vi "Autonomous Independent.vi"() -> ()   [LabVIEW 2020]
doc: "This VI is called when autonomous begins, and will automatically be terminated when autonomous ends. You can carry out timed or sensor driven robot movement independently without needing to return to the caller."
uses:
  <vilib>/Rock Robotics/WPI/ThirdParty/REV Robotics/REVLib/Typedef/Spark MAX Sensor Type.ctl
  <vilib>/Rock Robotics/WPI/Solenoid/WPI_SolenoidValue.ctl
  <vilib>/Rock Robotics/WPI/Utilities/WPI_GetSetVariantRefNum.vi
  <vilib>/Rock Robotics/Network Tables/NT Read String.vi
  <vilib>/Rock Robotics/Network Tables/NT Write Numeric Array.vi
  <vilib>/Rock Robotics/Network Tables/NT Write Number.vi
  Robot Global Data.vi
  <vilib>/Rock Robotics/WPI/Solenoid/WPI_SolenoidSetEnum.vi
  <vilib>/Rock Robotics/WPI/RobotDrive/WPI_RobotDriveArcadeDrive_Standard(NoSaturation).vi
panel:
  out "Right Drive Encoder 2":dbl format="%#.3f"
  out "Sensor Position 2":dbl
  out "Timestamp 2":u32
  out "Sensor Position":dbl
  out "Timestamp":u32
  in  "error in 2":errorcluster
  out "Real Yaw":dbl
  out "Right Drive Encoder":dbl format="%#.3f"
  in  "error in":errorcluster
  # "Be sure to right-click and choose Data Operations>>Make Current Value default if you want to save the array values with the VI"
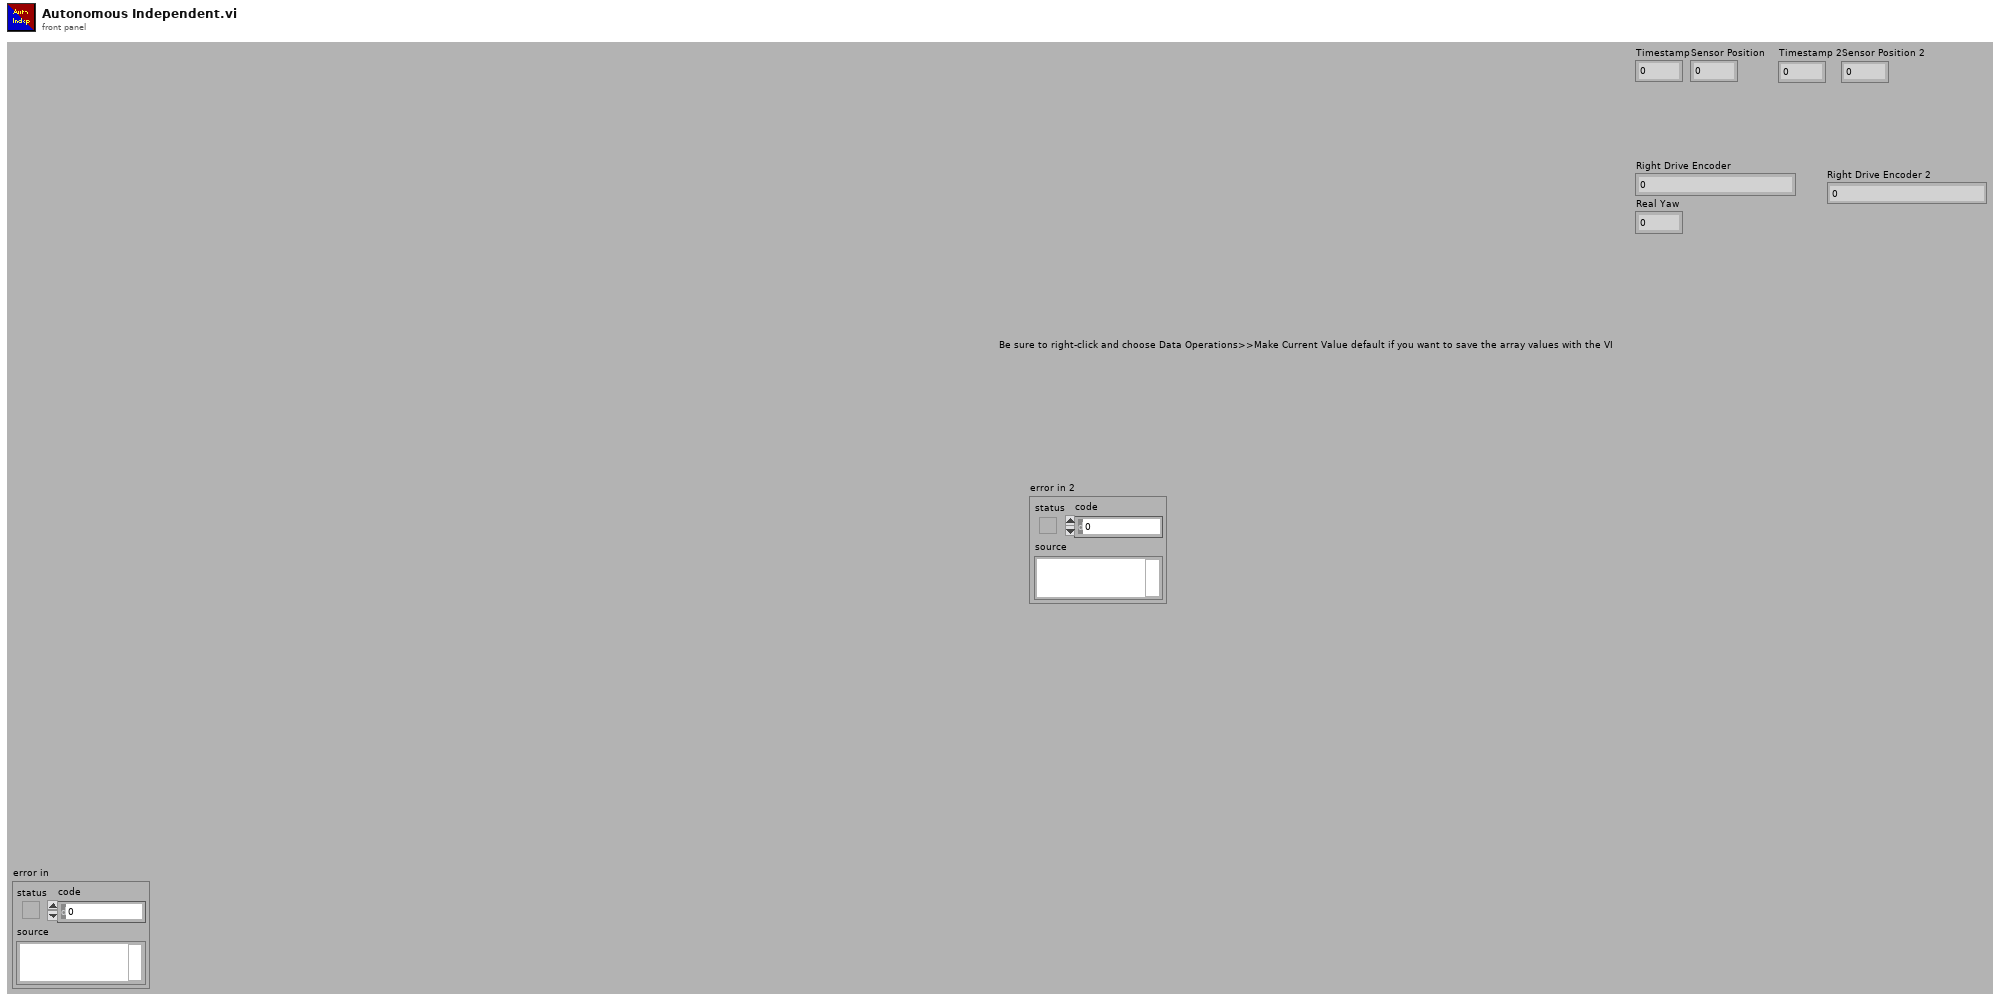
[diagram p1: front panel]
types:
  T1 = typedef "Spark MAX Sensor Type.ctl" = enum16{"No Sensor", "Hall Sensor", "Encoder", "-Not Available-", "Analog", "Alternate Encoder", "Duty Cycle"}
  T2 = typedef "WPI_JoystickDevRef.ctl" = cluster{"Device":T3}
  T3 = typedef "WPI_JoystickDeviceEnum.ctl" = enum16{"USB 0", "USB 1", "USB 2", "USB 3", "USB 4", "USB 5"}
  T4 = typedef "WPI_RobotDriveDevRef.ctl" = cluster{"DevStatus":errorcluster, "Motors[]":T5[], "Square Inputs":bool, "Max Output":dbl}
  T5 = typedef "WPI_MotorControlDeviceRef.ctl" = cluster{"DeviceStatus":errorcluster, "Type":T6, "PWM":cluster{"PWM Channel":T7, "DeadBand":T8}, "CAN":cluster{"Device Number":u8, "SetOutput VI Ref":variant, "GetOutput VI Ref":variant, "Enable VI Ref":variant, "Disable VI Ref":variant, "Data":variant}, "Invert":bool, "DIO PWM":cluster{"PWM \"Enable\" Channel":T7, "DIOChannel":T9, "PWM Rate":dbl}}
  T6 = typedef "WPI_MotorControlType.ctl" = enum16{"PWM", "CAN", "DIO PWM"}
  T7 = typedef "FPGA_DIOPWMChannel.ctl" = enum8{"PWM 0", "PWM 1", "PWM 2", "PWM 3", "PWM 4", "PWM 5", "PWM 6", "PWM 7", "PWM 8", "PWM 9", "PWM MXP 0", "PWM MXP 1", "PWM MXP 2", "PWM MXP 3", "PWM MXP 4", "PWM MXP 5", "PWM MXP 6", "PWM MXP 7", "PWM MXP 8", "PWM MXP 9", "Invalid"}
  T8 = typedef "WPI_PWMDeadband.ctl" = cluster{"Name":string, "maxPositivePwm":i32, "minPositivePwm":i32, "centerPwm":i32, "maxNegativePwm":i32, "minNegativePwm":i32, "angularRange":u16}
  T9 = typedef "FPGA_DIOChannel.ctl" = enum8{"DIO 0", "DIO 1", "DIO 2", "DIO 3", "DIO 4", "DIO 5", "DIO 6", "DIO 7", "DIO 8", "DIO 9", "DIO MXP 0", "DIO MXP 1", "DIO MXP 2", "DIO MXP 3", "DIO MXP 4", "DIO MXP 5", "DIO MXP 6", "DIO MXP 7", "DIO MXP 8", "DIO MXP 9", "DIO MXP 10", "DIO MXP 11", "DIO MXP 12", "DIO MXP 13", "DIO MXP 14", "DIO MXP 15", "SPI Port CS1", "SPI Port CS2", "SPI Port CS3", "SPI Port MISO", "SPI Port MOSI", "Invalid"}
  T10 = cluster{"Motors[][0]":T5, "Motors[][1]":T5, "Motors[][2]":T5, "Motors[][3]":T5, "Motors[][4]":T5, "Motors[][5]":T5, "Motors[][6]":T5, "Motors[][7]":T5, "Motors[][8]":T5}
  T11 = typedef "WPI_SolenoidValue.ctl" = enum16{"Off", "On", "Forward", "Reverse"}
  T12 = typedef "WPI_SolenoidDevRef.ctl" = cluster{"DevStatus":errorcluster, "Pneumatics Control Module":u8, "Forward Solenoid Channel":T13, "Reverse Solenoid Channel":T13}
  T13 = typedef "WPI_SolenoidChannel.ctl" = enum8{"Solenoid 0", "Solenoid 1", "Solenoid 2", "Solenoid 3", "Solenoid 4", "Solenoid 5", "Solenoid 6", "Solenoid 7", "Solenoid 8", "Solenoid 9", "Solenoid 10", "Solenoid 11", "Solenoid 12", "Solenoid 13", "Solenoid 14", "Solenoid 15", "Invalid"}
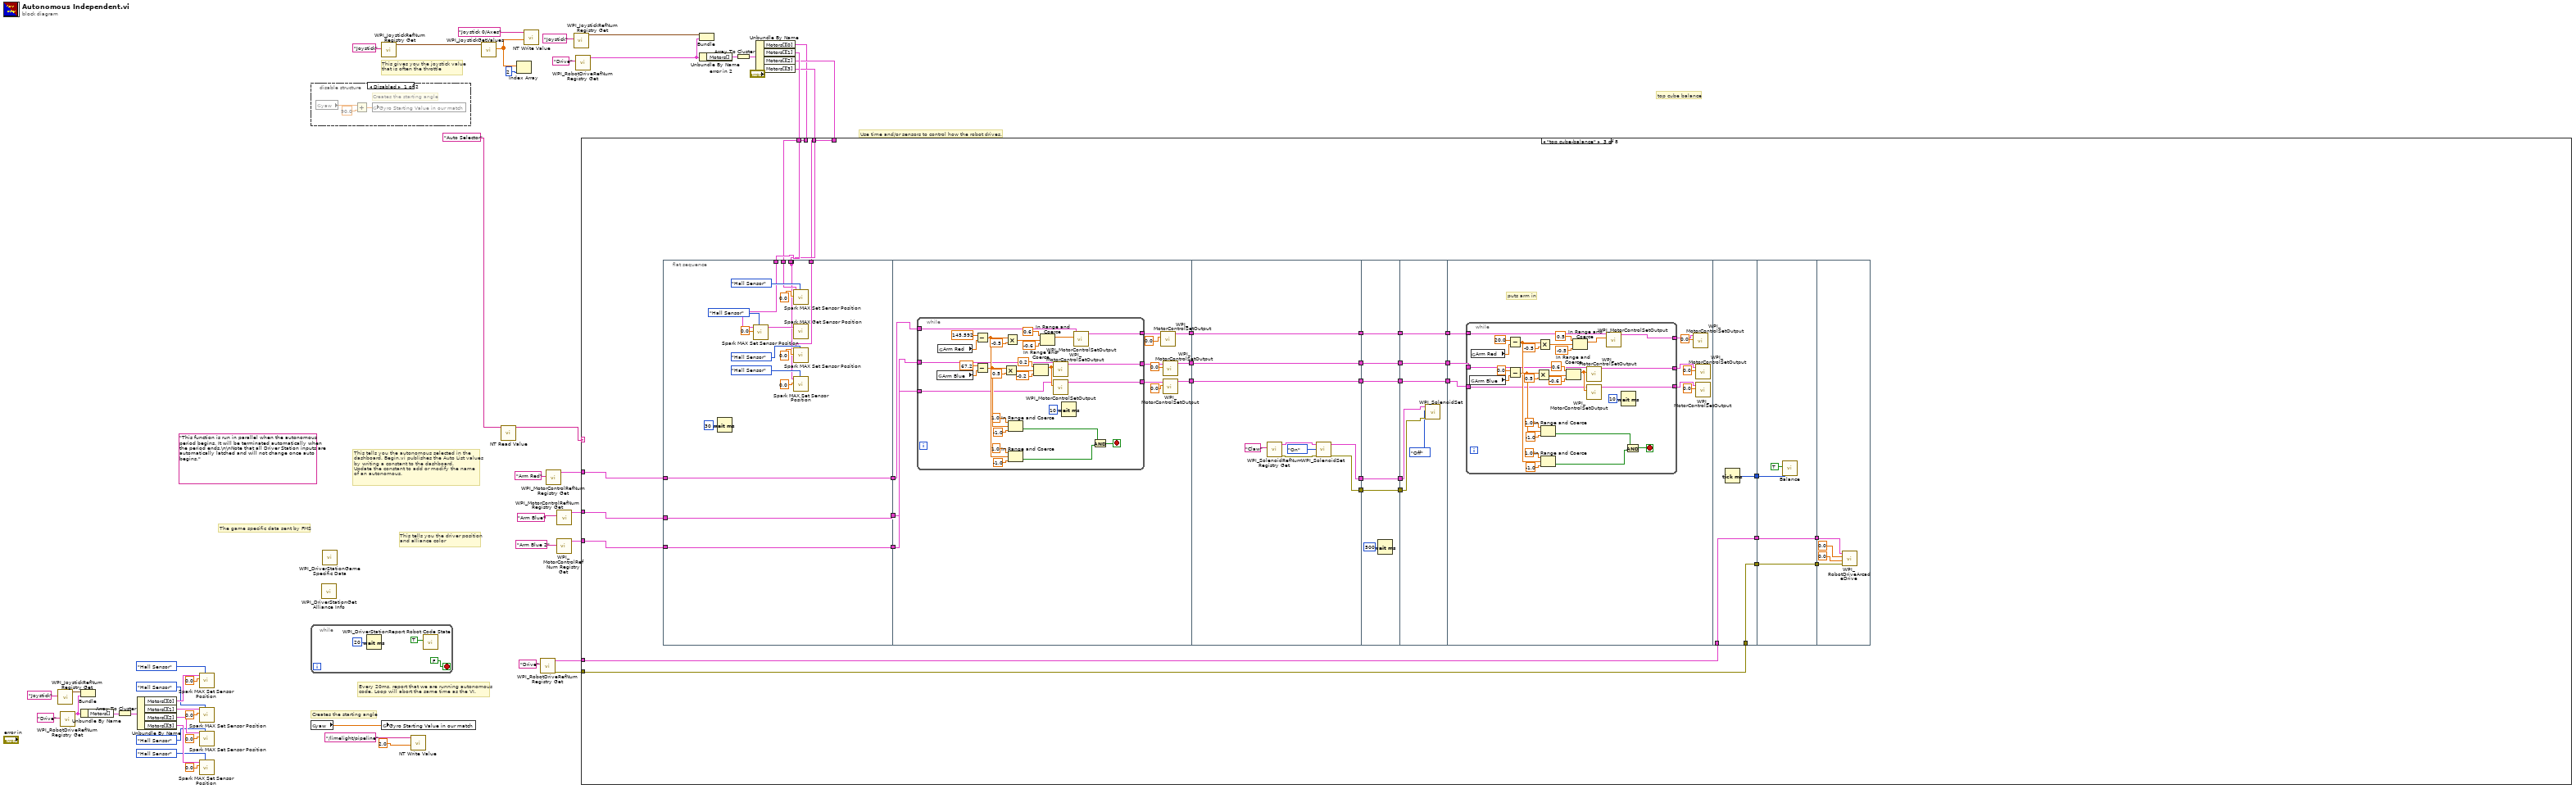
[diagram p0: block diagram]
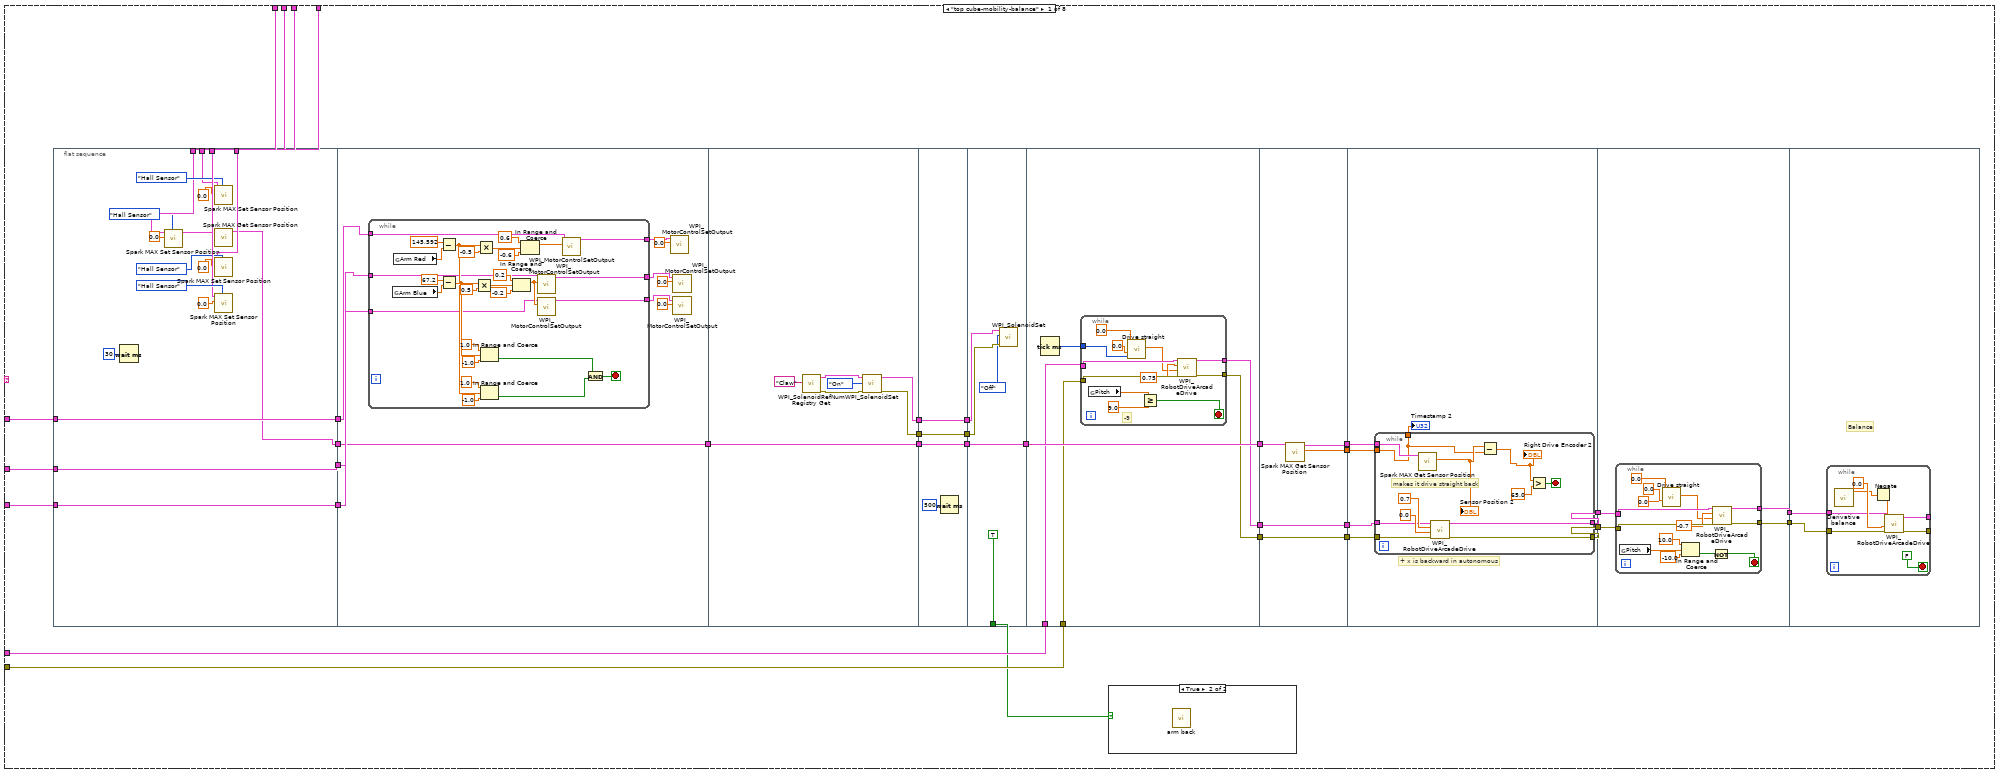
[diagram p3: hidden frame]
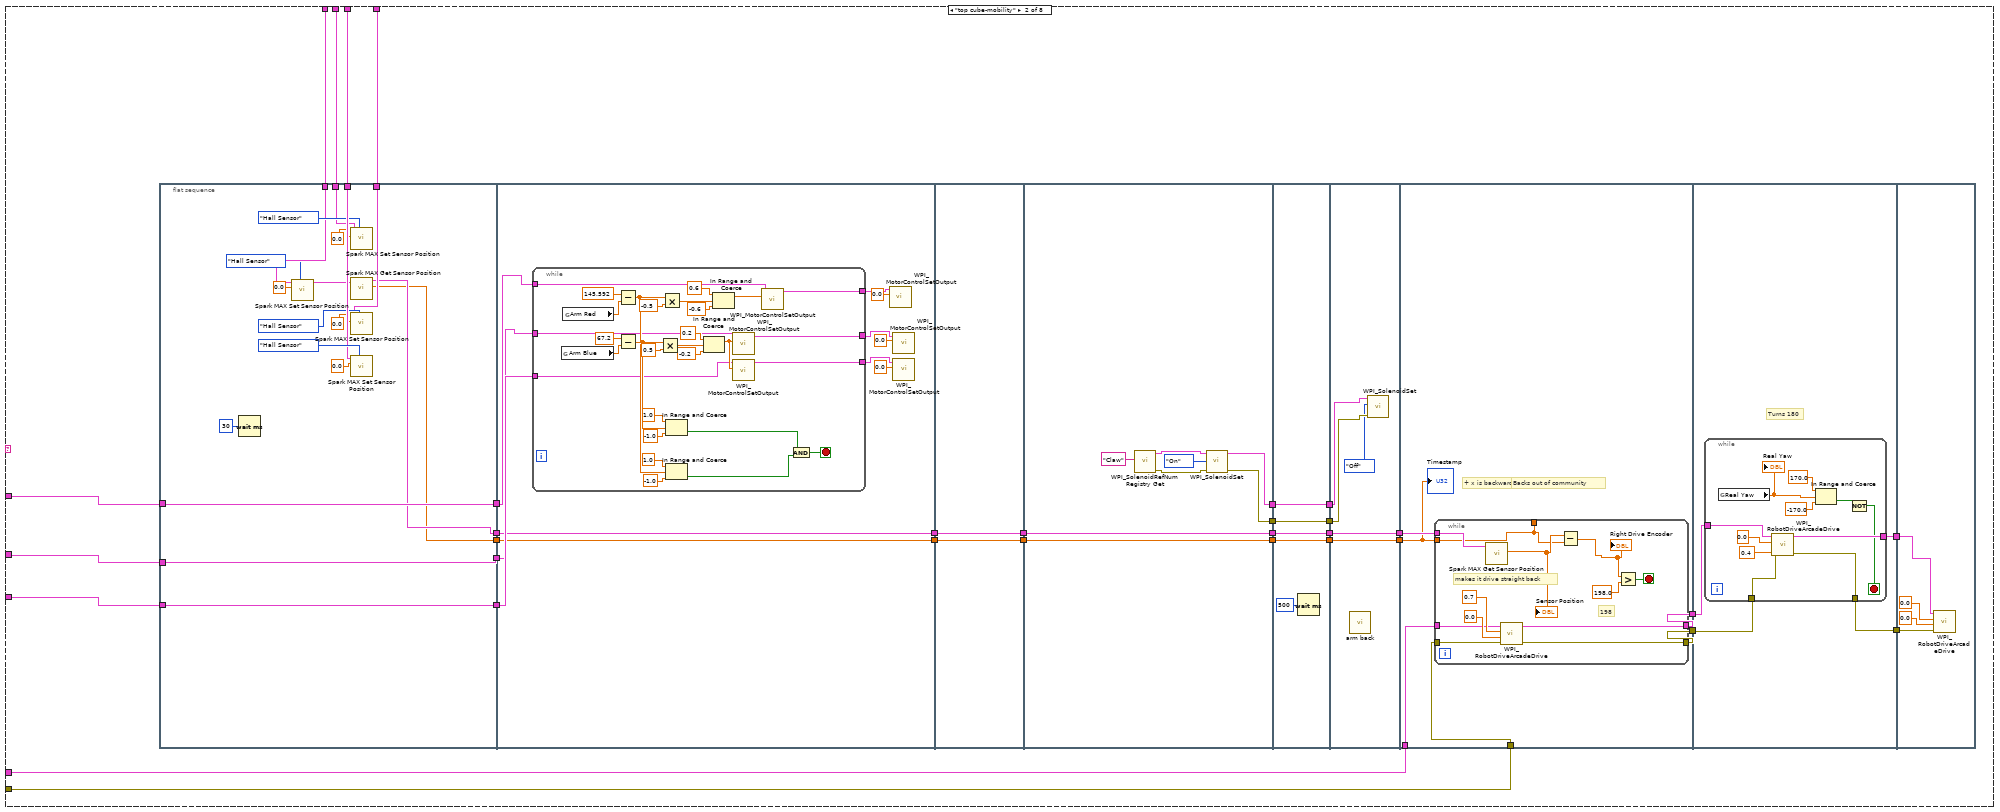
[diagram p5: hidden frame]
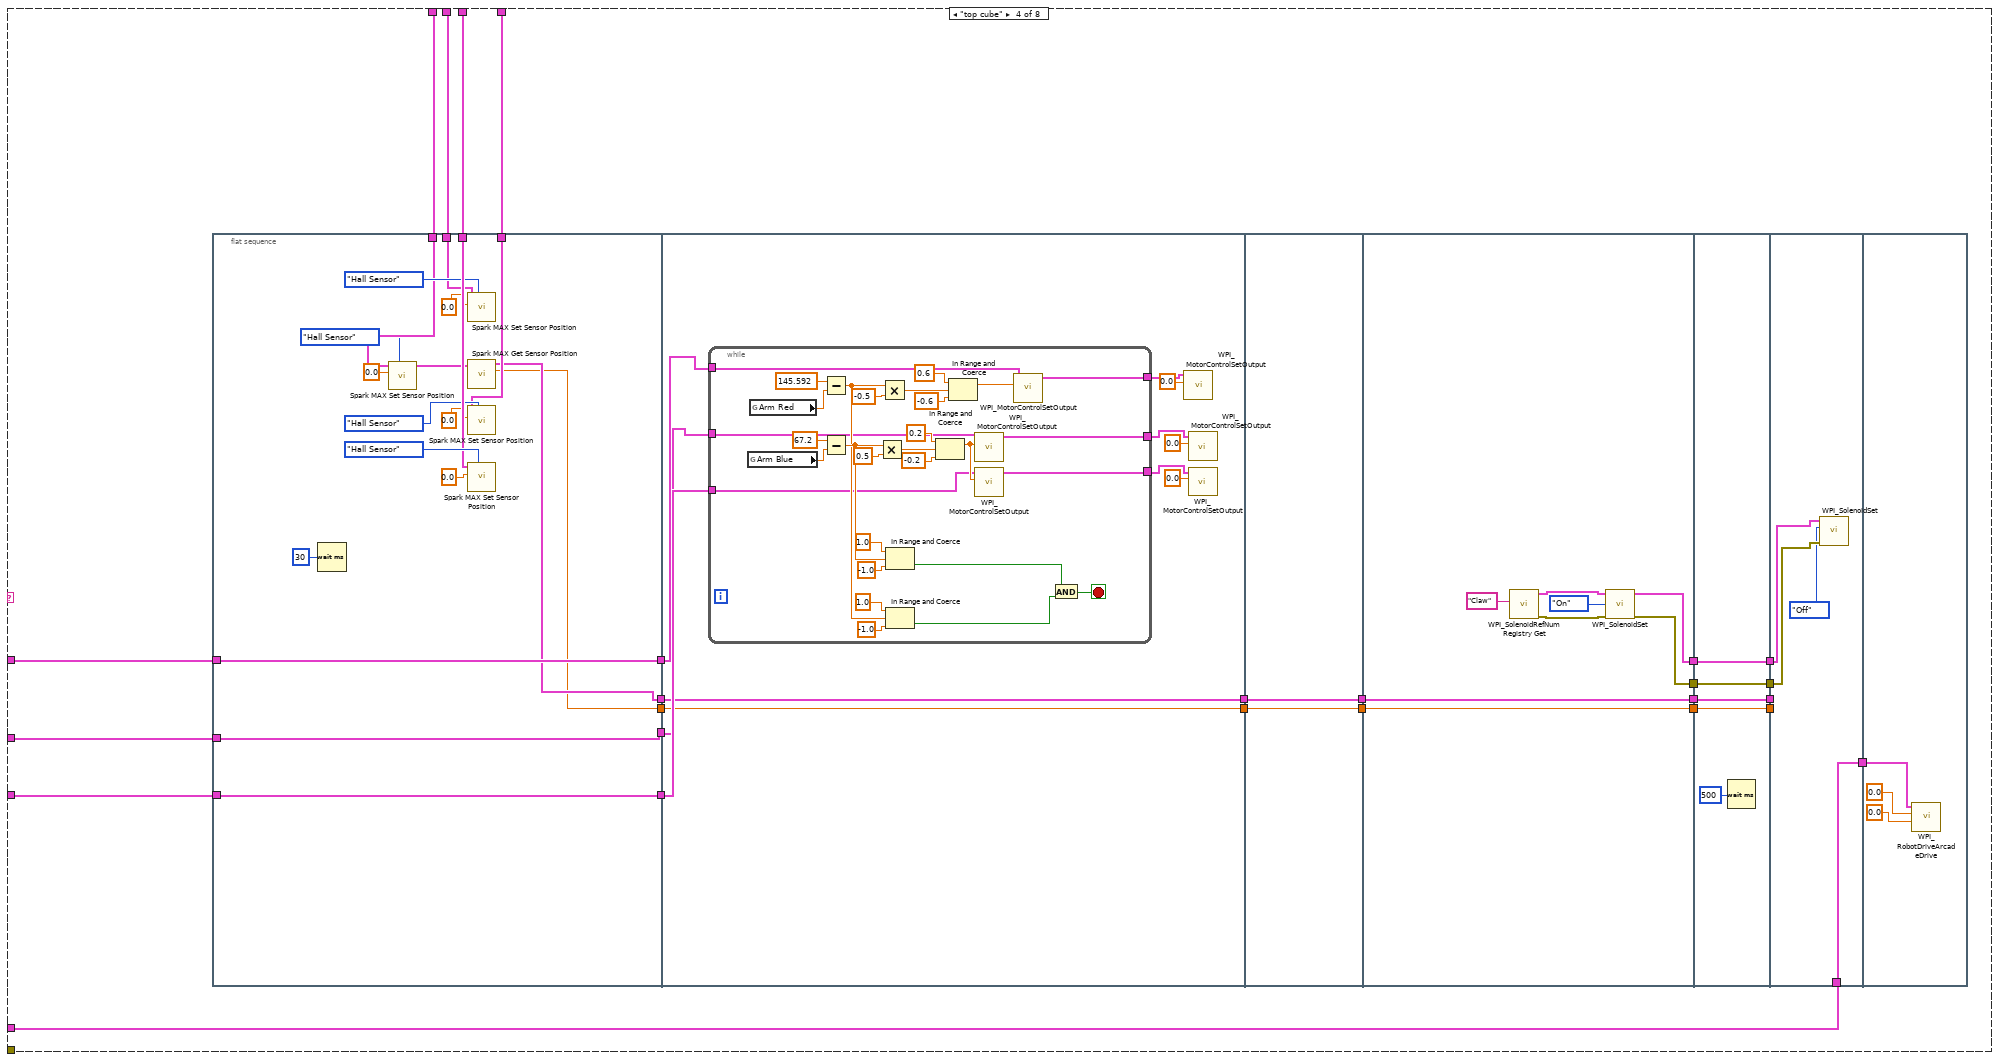
[diagram p6: hidden frame]
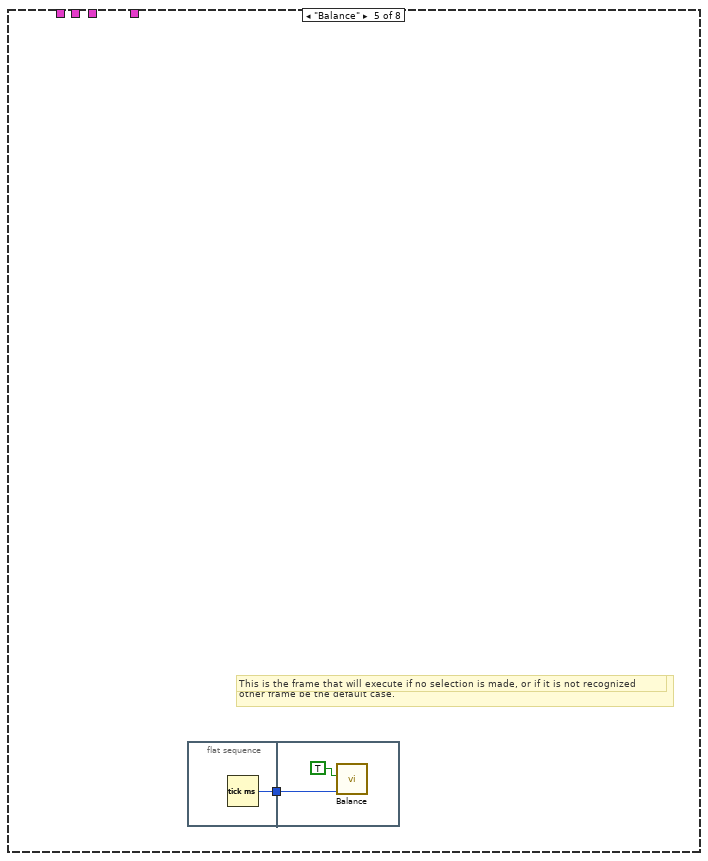
[diagram p7: hidden frame]
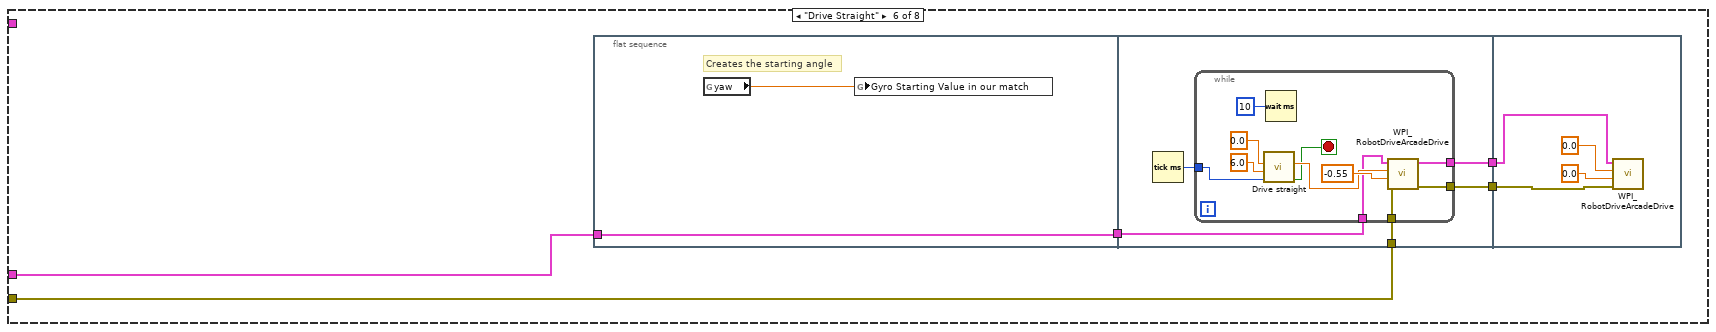
[diagram p8: hidden frame]
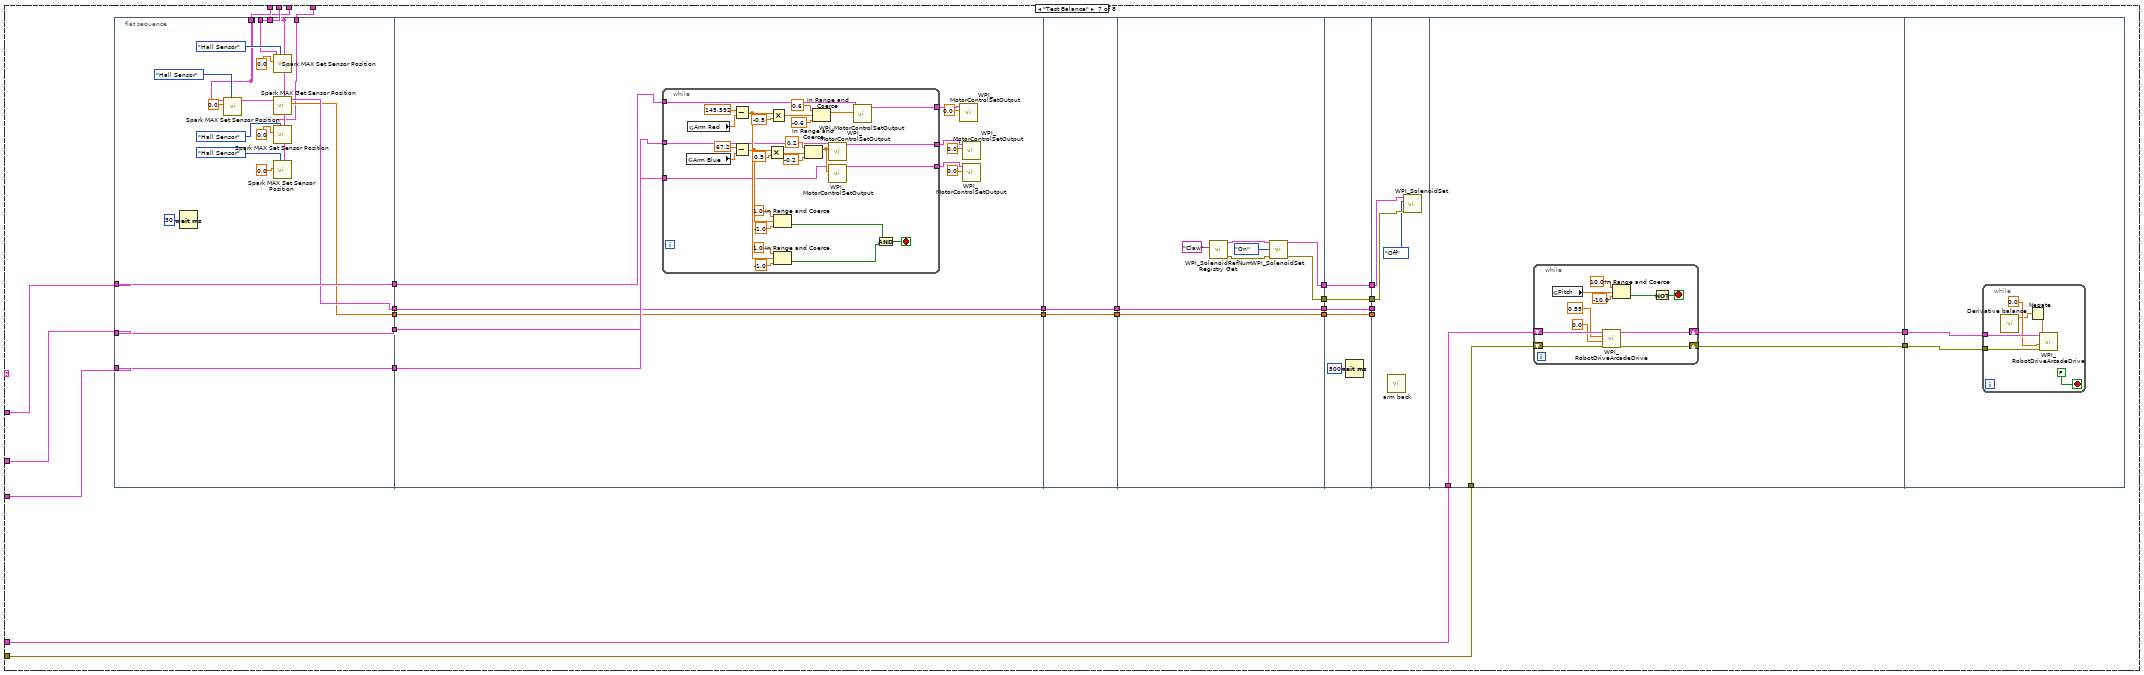
[diagram p9: hidden frame]
diagram:
  (unwired) "This function is run in parallel when the autonomous period begins. It will be terminated automatically when the period ends.\n\nNote that all Driver Station inputs are automatically latched and will not change once auto begins."
  # "top cube balance"
  # "Creates the starting angle"
  # "The game specific data sent by FMS"
  # "This tells you the autonomous selected in the \ndashboard. Begin.vi publishes the Auto List values\nby writing a constant to the dashboard.\nUpdate the constant to add or modify the name\nof an autonomous."
  # "Every 20ms, report that we are running autonomous\ncode. Loop will abort the same time as the VI."
  # "This gives you the joystick value\nthat is often the throttle"
  # "Use time and/or sensors to control how the robot drives."
  # "This tells you the driver position\nand alliance color"
  n1 = call <vilib>:"WPI_JoystickRefNum Registry Get.vi"("refnum name"="Joystick") -> ("JoystickDevRef"=w26:T2)  [unwired: 1 in, 9 out]
  n2 = call <vilib>:"WPI_RobotDriveRefNum Registry Get.vi"("refnum name"="Drive") -> ("RobotDriveDevRef"=w22:T4)  [unwired: 1 in, 9 out]
  n3 = Bundle("JoystickDevRef"=w26, "RobotDriveDevRef"=w22) -> ()  [unwired: 2 out]
  n4 = Unbundle By Name(w22) -> ("Motors[]"=w25:T5[])
  n5 = Array To Cluster(array=w25) -> (cluster=w24:T10)
  n6 = Unbundle By Name(w24) -> ("Motors[][0]"=w21:T5, "Motors[][1]"=w20:T5, "Motors[][2]"=w19:T5, "Motors[][3]"=w18:T5)
  n7 = call <vilib>:"Spark MAX Set Sensor Position.vi"("Sensor Type (Hall Sensor)"=Spark_MAX_Sensor_Type."Hall Sensor", "Position"=0.0, "MotorControlDeviceRef"=w21) -> ()  [unwired: 7 in, 2 out]
  n8 = call <vilib>:"Spark MAX Set Sensor Position.vi"("Sensor Type (Hall Sensor)"=Spark_MAX_Sensor_Type."Hall Sensor", "Position"=0.0, "MotorControlDeviceRef"=w20) -> ()  [unwired: 7 in, 2 out]
  n9 = call <vilib>:"Spark MAX Set Sensor Position.vi"("Sensor Type (Hall Sensor)"=Spark_MAX_Sensor_Type."Hall Sensor", "Position"=0.0, "MotorControlDeviceRef"=w19) -> ()  [unwired: 7 in, 2 out]
  n10 = call <vilib>:"Spark MAX Set Sensor Position.vi"("Sensor Type (Hall Sensor)"=Spark_MAX_Sensor_Type."Hall Sensor", "Position"=0.0, "MotorControlDeviceRef"=w18) -> ()  [unwired: 7 in, 2 out]
  n11 = disable-structure shown="Disabled" {
    frame Disabled {
      # "Creates the starting angle"
      n12 = global read "Robot Global Data.vi" "yaw"() -> (w49:dbl)
      n13 = Add(x=w49, y=90.0) -> (x+y=w50:dbl)
      n14 = global write "Robot Global Data.vi" "Gyro Starting Value in our match"(w50) -> ()
    }
    frame Enabled {
    }
  }
  n15 = while {
    stop <- FALSE stop-if-true
    n16 = Wait (ms)(milliseconds to wait=u32 20) -> ()  [unwired: 1 out]
    n17 = call <vilib>:"WPI_DriverStationReport Robot Code State.vi"("Autonomous"=TRUE) -> ()  [unwired: 10 in, 1 out]
  }
  n18 = global read "Robot Global Data.vi" "yaw"() -> (w40:dbl)
  n19 = call <vilib>:"WPI_DriverStationGet Alliance Info.vi"() -> ()  [unwired: 12 out]
  n20 = call <vilib>:"WPI_DriverStationGame Specific Data.vi"() -> ()  [unwired: 11 in, 1 out]
  n21 = call <vilib>:"WPI_JoystickRefNum Registry Get.vi"("refnum name"="Joystick") -> ("JoystickDevRef"=w46:T2)  [unwired: 1 in, 9 out]
  n22 = global write "Robot Global Data.vi" "Gyro Starting Value in our match"(w40) -> ()
  n23 = call-poly <vilib>:"NT Write Value.vi"("value"=2.0, "name"="/limelight/pipeline" ("Name")) -> ()  [unwired: 9 in, 1 out]
  n24 = call <vilib>:"WPI_JoystickGetValues.vi"("JoystickDevRef"=w46) -> ("Axes"=w42:dbl[])  [unwired: 6 in, 4 out]
  n25 = call-poly <vilib>:"NT Read Value.vi"("name"="Auto Selector" ("Name")) -> ("value"=w43:string)  [unwired: 8 in, 2 out]
  n26 = Index Array(array=w42, index=2) -> ()  [unwired: 1 out]
  n27 = call-poly <vilib>:"NT Write Value.vi"("value"=w42, "name"="Joystick 0/Axes" ("Name")) -> ()  [unwired: 9 in, 1 out]
  n28 = call <vilib>:"WPI_RobotDriveRefNum Registry Get.vi"("refnum name"="Drive") -> ("error out"=w29:errorcluster, "RobotDriveDevRef"=w30:T4)  [unwired: 9 in]
  n29 = call <vilib>:"WPI_MotorControlRefNum Registry Get.vi"("refnum name"="Arm Red") -> ("MotorControlDevRef"=w34:T5)  [unwired: 9 in, 1 out]
  n30 = call <vilib>:"WPI_MotorControlRefNum Registry Get.vi"("refnum name"="Arm Blue 2") -> ("MotorControlDevRef"=w32:T5)  [unwired: 9 in, 1 out]
  n31 = call <vilib>:"WPI_MotorControlRefNum Registry Get.vi"("refnum name"="Arm Blue") -> ("MotorControlDevRef"=w33:T5)  [unwired: 9 in, 1 out]
  n32 = call <vilib>:"WPI_JoystickRefNum Registry Get.vi"("refnum name"="Joystick") -> ("JoystickDevRef"=w7:T2)  [unwired: 1 in, 9 out]
  n33 = call <vilib>:"WPI_RobotDriveRefNum Registry Get.vi"("refnum name"="Drive") -> ("RobotDriveDevRef"=w10:T4)  [unwired: 1 in, 9 out]
  n34 = Bundle("JoystickDevRef"=w7, "RobotDriveDevRef"=w10) -> ()  [unwired: 2 out]
  n35 = Unbundle By Name(w10) -> ("Motors[]"=w8:T5[])
  n36 = Array To Cluster(array=w8) -> (cluster=w9:T10)
  n37 = Unbundle By Name(w9) -> ("Motors[][0]"=w1:T5, "Motors[][1]"=w4:T5, "Motors[][2]"=w2:T5, "Motors[][3]"=w3:T5)
  n38 = case shown="\"top cube-balance\"" w43 {
    tunnel: w34 -> [w86 w261 w403 w566 _ _ w685 _]
    tunnel: w33 -> [w85 w260 w402 w565 _ _ w684 _]
    tunnel: w32 -> [w84 w259 w401 w564 _ _ w683 _]
    tunnel: w30 -> [w68 w254 w400 w541 _ w653 w682 _]
    tunnel: w29 -> [w67 w253 w399 _ _ w652 w681 _]
    tunnel: w4 -> [w73 w239 w397 w551 _ _ w689 _]
    tunnel: w3 -> [w72 w238 w395 w550 _ _ w687 _]
    tunnel: w2 -> [w71 w237 w394 w549 _ _ w686 _]
    tunnel: w1 -> [w70 w236 w396 w548 _ _ w688 _]
    frame "top cube-mobility-balance" {
      n39 = flat-sequence {
        tunnel: w84 -> [w104]
        tunnel: w85 -> [w103]
        tunnel: w86 -> [w102]
        tunnel: [w104] -> w79
        tunnel: [w92] -> w76
        tunnel: [w103] -> w75
        tunnel: [w102] -> w74
        tunnel: w73 -> [w90]
        tunnel: w72 -> [w99]
        tunnel: w71 -> [w96]
        tunnel: w70 -> [w93]
        tunnel: w79 -> [w114]
        tunnel: [w113] -> w55
        tunnel: w76 -> [w113]
        tunnel: w75 -> [w111]
        tunnel: w74 -> [w112]
        tunnel: [w150] -> w83
        tunnel: [w149] -> w81
        tunnel: [w148] -> w77
        tunnel: w55 -> [w148]
        tunnel: w83 -> [w154]
        tunnel: [w154] -> w82
        tunnel: w81 -> [w153]
        tunnel: [w153] -> w80
        tunnel: [w152] -> w78
        tunnel: w77 -> [w152]
        tunnel: w82 -> [w159]
        tunnel: w80 -> [w158]
        tunnel: [w157] -> w69
        tunnel: w78 -> [w157]
        tunnel: [TRUE] -> w54
        tunnel: w69 -> [w165]
        tunnel: [w165] -> w64
        tunnel: w68 -> [w163]
        tunnel: w67 -> [w162]
        tunnel: [w161] -> w62
        tunnel: [w160] -> w60
        tunnel: w64 -> [w180]
        tunnel: [w179] -> w63
        tunnel: w62 -> [w182]
        tunnel: [w182] -> w61
        tunnel: w60 -> [w181]
        tunnel: [w181] -> w59
        tunnel: [w178] -> w58
        tunnel: [w189] -> w66
        tunnel: [w188] -> w65
        tunnel: w63 -> [w187]
        tunnel: w61 -> [w186]
        tunnel: w59 -> [w185]
        tunnel: w58 -> [w184]
        tunnel: w66 -> [w205]
        tunnel: [w203] -> w57
        tunnel: w65 -> [w204]
        tunnel: [w202] -> w56
        tunnel: w57 -> [w221]
        tunnel: w56 -> [w220]
        frame #0 {
          n40 = Wait (ms)(milliseconds to wait=u32 30) -> ()  [unwired: 1 out]
          n41 = call <vilib>:"Spark MAX Set Sensor Position.vi"("Sensor Type (Hall Sensor)"=Spark_MAX_Sensor_Type."Hall Sensor", "Position"=0.0, "MotorControlDeviceRef"=w90) -> ("MotorControlDeviceRef"=w89:T5)  [unwired: 7 in, 1 out]
          n42 = call <vilib>:"Spark MAX Set Sensor Position.vi"("Sensor Type (Hall Sensor)"=Spark_MAX_Sensor_Type."Hall Sensor", "Position"=0.0, "MotorControlDeviceRef"=w93) -> ()  [unwired: 7 in, 2 out]
          n43 = call <vilib>:"Spark MAX Get Sensor Position.vi"("MotorControlDevRef in"=w89) -> ("MotorControlDevRef out"=w92:T5)  [unwired: 7 in, 3 out]
          n44 = call <vilib>:"Spark MAX Set Sensor Position.vi"("Sensor Type (Hall Sensor)"=Spark_MAX_Sensor_Type."Hall Sensor", "Position"=0.0, "MotorControlDeviceRef"=w96) -> ()  [unwired: 7 in, 2 out]
          n45 = call <vilib>:"Spark MAX Set Sensor Position.vi"("Sensor Type (Hall Sensor)"=Spark_MAX_Sensor_Type."Hall Sensor", "Position"=0.0, "MotorControlDeviceRef"=w99) -> ()  [unwired: 7 in, 2 out]
        }
        frame #1 {
          n46 = while {
            tunnel: w112 -> [w120]
            tunnel: w111 -> [w119]
            tunnel: w114 -> [w118]
            tunnel: [w115] -> w110
            tunnel: [w117] -> w109
            tunnel: [w116] -> w108
            stop <- w143 stop-if-true
            n47 = global read "Robot Global Data.vi" "Arm Blue"() -> (w123:dbl)
            n48 = global read "Robot Global Data.vi" "Arm Red"() -> (w134:dbl)
            n49 = Subtract(x=145.592, y=w134) -> (x-y=w121:dbl)
            n50 = Subtract(x=67.2, y=w123) -> (x-y=w122:dbl)
            n51 = Multiply(x=w122, y=0.5) -> (x*y=w131:dbl)
            n52 = Multiply(x=w121, y=-0.5) -> (x*y=w130:dbl)
            n53 = In Range and Coerce(upper limit=1.0, x=w122, lower limit=-1.0) -> (In Range?=w142:bool)  [unwired: 1 out]
            n54 = In Range and Coerce(upper limit=1.0, x=w121, lower limit=-1.0) -> (In Range?=w141:bool)  [unwired: 1 out]
            n55 = In Range and Coerce(upper limit=0.2, x=w131, lower limit=-0.2) -> (coerced(x)=w126:dbl)  [unwired: 1 out]
            n56 = In Range and Coerce(upper limit=0.6, x=w130, lower limit=-0.6) -> (coerced(x)=w127:dbl)  [unwired: 1 out]
            n57 = call <vilib>:"WPI_MotorControlSetOutput.vi"("Output"=w126, "MotorControlDevRef"=w119) -> ("MotorControlDevRef"=w115:T5)  [unwired: 7 in, 2 out]
            n58 = call <vilib>:"WPI_MotorControlSetOutput.vi"("Output"=w126, "MotorControlDevRef"=w118) -> ("MotorControlDevRef"=w117:T5)  [unwired: 7 in, 2 out]
            n59 = call <vilib>:"WPI_MotorControlSetOutput.vi"("Output"=w127, "MotorControlDevRef"=w120) -> ("MotorControlDevRef"=w116:T5)  [unwired: 7 in, 2 out]
            n60 = And(x=w142, y=w141) -> (x .and. y?=w143:bool)
          }
          n61 = call <vilib>:"WPI_MotorControlSetOutput.vi"("Output"=0.0, "MotorControlDevRef"=w108) -> ()  [unwired: 7 in, 3 out]
          n62 = call <vilib>:"WPI_MotorControlSetOutput.vi"("Output"=0.0, "MotorControlDevRef"=w110) -> ()  [unwired: 7 in, 3 out]
          n63 = call <vilib>:"WPI_MotorControlSetOutput.vi"("Output"=0.0, "MotorControlDevRef"=w109) -> ()  [unwired: 7 in, 3 out]
        }
        frame #2 {
          n64 = call <vilib>:"WPI_SolenoidRefNum Registry Get.vi"("refnum name"="Claw") -> ("error out"=w147:errorcluster, "SolenoidDevRef"=w146:T12)  [unwired: 9 in]
          n65 = call-poly <vilib>:"WPI_SolenoidSet.vi"("error in (no error)"=w147, "Value"=WPI_SolenoidValue."On", "SolenoidDevRef"=w146) -> ("error out"=w149:errorcluster, "SolenoidDevRef"=w150:T12)  [unwired: 7 in]
        }
        frame #3 {
          n66 = Wait (ms)(milliseconds to wait=u32 500) -> ()  [unwired: 1 out]
        }
        frame #4 {
          n67 = call-poly <vilib>:"WPI_SolenoidSet.vi"("error in (no error)"=w158, "Value"=WPI_SolenoidValue."Off", "SolenoidDevRef"=w159) -> ()  [unwired: 7 in, 2 out]
        }
        frame #5 {
          n68 = Tick Count (ms)() -> (millisecond timer value=w164:u32)
          n69 = while {
            tunnel: [w175] -> w161
            tunnel: w163 -> [w174]
            tunnel: w162 -> [w173]
            tunnel: [w171] -> w160
            tunnel: w164 -> [w167]
            stop <- w177 stop-if-true
            # "-9"
            n70 = global read "Robot Global Data.vi" "Pitch"() -> (w172:dbl)
            n71 = call "Drive straight.vi"("Start Time"=w167, "Length(seconds)"=0.0, "Desired angle"=0.0) -> ("X Power"=w168:dbl)  [unwired: 7 in, 1 out]
            n72 = Greater Or Equal?(x=w172, y=9.0) -> (x >= y?=w177:bool)
            n73 = call-poly <vilib>:"WPI_RobotDriveArcadeDrive.vi"("error in (no error)"=w173, "Y axis value"=w168, "X axis value"=0.75 ("Y axis value"), "RobotDriveDevRef"=w174) -> ("error out"=w171:errorcluster, "RobotDriveDevRef"=w175:T4)  [unwired: 5 in, 1 out]
          }
        }
        frame #6 {
          n74 = call <vilib>:"Spark MAX Get Sensor Position.vi"("MotorControlDevRef in"=w180) -> ("Sensor Position"=w178:dbl, "MotorControlDevRef out"=w179:T5)  [unwired: 7 in, 2 out]
        }
        frame #7 {
          # "+ x is backward in autonomous"
          n75 = while {
            tunnel: [w199] -> w189
            tunnel: [w198] -> w188
            tunnel: w186 -> [w196]
            tunnel: w187 -> [w194]
            tunnel: w185 -> [w191]
            tunnel: w184 -> [w190]
            tunnel: [w190] -> w183
            stop <- w197 stop-if-true
            # "makes it drive straight back"
            n76 = call <vilib>:"Spark MAX Get Sensor Position.vi"("MotorControlDevRef in"=w194) -> ("Sensor Position"=w192:dbl)  [unwired: 7 in, 3 out]
            "Sensor Position 2" <- w192
            n77 = call-poly <vilib>:"WPI_RobotDriveArcadeDrive.vi"("error in (no error)"=w191, "Y axis value"=0.0, "X axis value"=0.7, "RobotDriveDevRef"=w196) -> ("error out"=w198:errorcluster, "RobotDriveDevRef"=w199:T4)  [unwired: 5 in, 1 out]
            n78 = Subtract(x=w192, y=w190) -> (x-y=w193:dbl)
            "Right Drive Encoder 2" <- w193
            n79 = Greater?(x=w193, y=65.0) -> (0:w197:bool)
          }
          "Timestamp 2" <- w183
        }
        frame #8 {
          n80 = while {
            tunnel: [w219] -> w203
            tunnel: w205 -> [w218]
            tunnel: w204 -> [w217]
            tunnel: [w216] -> w202
            stop <- w206 stop-if-true
            n81 = global read "Robot Global Data.vi" "Pitch"() -> (w208:dbl)
            n82 = call "Drive straight.vi"("Start Time"=0.0, "Length(seconds)"=0.0, "Desired angle"=0.0) -> ("X Power"=w213:dbl)  [unwired: 7 in, 1 out]
            n83 = In Range and Coerce(upper limit=10.0, x=w208, lower limit=-10.0 ("y")) -> (In Range?=w209:bool)  [unwired: 1 out]
            n84 = Not(x=w209) -> (.not. x?=w206:bool)
            n85 = call-poly <vilib>:"WPI_RobotDriveArcadeDrive.vi"("error in (no error)"=w217, "Y axis value"=w213, "X axis value"=-0.7 ("Y axis value"), "RobotDriveDevRef"=w218) -> ("error out"=w216:errorcluster, "RobotDriveDevRef"=w219:T4)  [unwired: 5 in, 1 out]
          }
        }
        frame #9 {
          # "Balance"
          n86 = while {
            tunnel: w221 -> [w225]
            tunnel: w220 -> [w224]
            tunnel: [w223] -> _
            tunnel: [w222] -> _
            stop <- FALSE stop-if-true
            n87 = call "Derivative balance.vi"() -> ("Motor Power"=w227:dbl)  [unwired: 11 in]
            n88 = Negate(x=w227) -> (-x=w226:dbl)
            n89 = call-poly <vilib>:"WPI_RobotDriveArcadeDrive.vi"("error in (no error)"=w224, "Y axis value"=0.0 ("X axis value"), "X axis value"=w226, "RobotDriveDevRef"=w225) -> ("error out"=w222:errorcluster, "RobotDriveDevRef"=w223:T4)  [unwired: 5 in, 1 out]
          }
        }
      }
      n90 = case shown="True" w54 {
        frame False {
        }
        frame True {
          n91 = call "arm back.vi"() -> ()  [unwired: 12 in]
        }
      }
    }
    frame "top cube-mobility" {
      n92 = flat-sequence {
        tunnel: w259 -> [w280]
        tunnel: w260 -> [w279]
        tunnel: w261 -> [w278]
        tunnel: [w280] -> w248
        tunnel: [w268] -> w242
        tunnel: [w279] -> w241
        tunnel: [w278] -> w240
        tunnel: w239 -> [w265]
        tunnel: w238 -> [w275]
        tunnel: w237 -> [w272]
        tunnel: w236 -> [w269]
        tunnel: [w267] -> w230
        tunnel: w248 -> [w291]
        tunnel: [w290] -> w243
        tunnel: w242 -> [w290]
        tunnel: w241 -> [w288]
        tunnel: w240 -> [w289]
        tunnel: [w287] -> w231
        tunnel: w230 -> [w287]
        tunnel: [w322] -> w244
        tunnel: w243 -> [w322]
        tunnel: [w321] -> w232
        tunnel: w231 -> [w321]
        tunnel: [w330] -> w258
        tunnel: [w329] -> w256
        tunnel: [w328] -> w245
        tunnel: w244 -> [w328]
        tunnel: [w327] -> w233
        tunnel: w232 -> [w327]
        tunnel: w258 -> [w335]
        tunnel: [w335] -> w257
        tunnel: w256 -> [w334]
        tunnel: [w334] -> w255
        tunnel: [w333] -> w246
        tunnel: w245 -> [w333]
        tunnel: [w332] -> w234
        tunnel: w233 -> [w332]
        tunnel: w257 -> [w340]
        tunnel: w255 -> [w339]
        tunnel: [w338] -> w247
        tunnel: w246 -> [w338]
        tunnel: [w337] -> w235
        tunnel: w234 -> [w337]
        tunnel: [w346] -> w252
        tunnel: [w345] -> w251
        tunnel: w254 -> [w344]
        tunnel: w253 -> [w343]
        tunnel: w247 -> [w342]
        tunnel: w235 -> [w341]
        tunnel: w252 -> [w362]
        tunnel: w251 -> [w361]
        tunnel: [w360] -> w250
        tunnel: [w359] -> w249
        tunnel: w250 -> [w375]
        tunnel: w249 -> [w374]
        frame #0 {
          n93 = Wait (ms)(milliseconds to wait=u32 30) -> ()  [unwired: 1 out]
          n94 = call <vilib>:"Spark MAX Set Sensor Position.vi"("Sensor Type (Hall Sensor)"=Spark_MAX_Sensor_Type."Hall Sensor", "Position"=0.0, "MotorControlDeviceRef"=w265) -> ("MotorControlDeviceRef"=w264:T5)  [unwired: 7 in, 1 out]
          n95 = call <vilib>:"Spark MAX Set Sensor Position.vi"("Sensor Type (Hall Sensor)"=Spark_MAX_Sensor_Type."Hall Sensor", "Position"=0.0, "MotorControlDeviceRef"=w269) -> ()  [unwired: 7 in, 2 out]
          n96 = call <vilib>:"Spark MAX Get Sensor Position.vi"("MotorControlDevRef in"=w264) -> ("Sensor Position"=w267:dbl, "MotorControlDevRef out"=w268:T5)  [unwired: 7 in, 2 out]
          n97 = call <vilib>:"Spark MAX Set Sensor Position.vi"("Sensor Type (Hall Sensor)"=Spark_MAX_Sensor_Type."Hall Sensor", "Position"=0.0, "MotorControlDeviceRef"=w272) -> ()  [unwired: 7 in, 2 out]
          n98 = call <vilib>:"Spark MAX Set Sensor Position.vi"("Sensor Type (Hall Sensor)"=Spark_MAX_Sensor_Type."Hall Sensor", "Position"=0.0, "MotorControlDeviceRef"=w275) -> ()  [unwired: 7 in, 2 out]
        }
        frame #1 {
          n99 = while {
            tunnel: w289 -> [w297]
            tunnel: w288 -> [w296]
            tunnel: w291 -> [w295]
            tunnel: [w292] -> w286
            tunnel: [w294] -> w285
            tunnel: [w293] -> w284
            stop <- w320 stop-if-true
            n100 = global read "Robot Global Data.vi" "Arm Blue"() -> (w300:dbl)
            n101 = global read "Robot Global Data.vi" "Arm Red"() -> (w311:dbl)
            n102 = Subtract(x=145.592, y=w311) -> (x-y=w298:dbl)
            n103 = Subtract(x=67.2, y=w300) -> (x-y=w299:dbl)
            n104 = Multiply(x=w299, y=0.5) -> (x*y=w308:dbl)
            n105 = Multiply(x=w298, y=-0.5) -> (x*y=w307:dbl)
            n106 = In Range and Coerce(upper limit=1.0, x=w299, lower limit=-1.0) -> (In Range?=w319:bool)  [unwired: 1 out]
            n107 = In Range and Coerce(upper limit=1.0, x=w298, lower limit=-1.0) -> (In Range?=w318:bool)  [unwired: 1 out]
            n108 = In Range and Coerce(upper limit=0.2, x=w308, lower limit=-0.2) -> (coerced(x)=w303:dbl)  [unwired: 1 out]
            n109 = In Range and Coerce(upper limit=0.6, x=w307, lower limit=-0.6) -> (coerced(x)=w304:dbl)  [unwired: 1 out]
            n110 = call <vilib>:"WPI_MotorControlSetOutput.vi"("Output"=w303, "MotorControlDevRef"=w296) -> ("MotorControlDevRef"=w292:T5)  [unwired: 7 in, 2 out]
            n111 = call <vilib>:"WPI_MotorControlSetOutput.vi"("Output"=w303, "MotorControlDevRef"=w295) -> ("MotorControlDevRef"=w294:T5)  [unwired: 7 in, 2 out]
            n112 = call <vilib>:"WPI_MotorControlSetOutput.vi"("Output"=w304, "MotorControlDevRef"=w297) -> ("MotorControlDevRef"=w293:T5)  [unwired: 7 in, 2 out]
            n113 = And(x=w319, y=w318) -> (x .and. y?=w320:bool)
          }
          n114 = call <vilib>:"WPI_MotorControlSetOutput.vi"("Output"=0.0, "MotorControlDevRef"=w284) -> ()  [unwired: 7 in, 3 out]
          n115 = call <vilib>:"WPI_MotorControlSetOutput.vi"("Output"=0.0, "MotorControlDevRef"=w286) -> ()  [unwired: 7 in, 3 out]
          n116 = call <vilib>:"WPI_MotorControlSetOutput.vi"("Output"=0.0, "MotorControlDevRef"=w285) -> ()  [unwired: 7 in, 3 out]
        }
        frame #2 {
        }
        frame #3 {
          n117 = call <vilib>:"WPI_SolenoidRefNum Registry Get.vi"("refnum name"="Claw") -> ("error out"=w326:errorcluster, "SolenoidDevRef"=w325:T12)  [unwired: 9 in]
          n118 = call-poly <vilib>:"WPI_SolenoidSet.vi"("error in (no error)"=w326, "Value"=WPI_SolenoidValue."On", "SolenoidDevRef"=w325) -> ("error out"=w329:errorcluster, "SolenoidDevRef"=w330:T12)  [unwired: 7 in]
        }
        frame #4 {
          n119 = Wait (ms)(milliseconds to wait=u32 500) -> ()  [unwired: 1 out]
        }
        frame #5 {
          n120 = call "arm back.vi"() -> ()  [unwired: 12 in]
          n121 = call-poly <vilib>:"WPI_SolenoidSet.vi"("error in (no error)"=w339, "Value"=WPI_SolenoidValue."Off", "SolenoidDevRef"=w340) -> ()  [unwired: 7 in, 2 out]
        }
        frame #6 {
          # "Backs out of community"
          # "+ x is backward in autonomous"
          n122 = while {
            tunnel: [w356] -> w346
            tunnel: [w355] -> w345
            tunnel: w344 -> [w353]
            tunnel: w343 -> [w352]
            tunnel: w342 -> [w350]
            tunnel: w341 -> [w347]
            tunnel: [w347] -> _
            stop <- w354 stop-if-true
            # "198"
            # "makes it drive straight back"
            n123 = call <vilib>:"Spark MAX Get Sensor Position.vi"("MotorControlDevRef in"=w350) -> ("Sensor Position"=w348:dbl)  [unwired: 7 in, 3 out]
            "Sensor Position" <- w348
            n124 = call-poly <vilib>:"WPI_RobotDriveArcadeDrive.vi"("error in (no error)"=w352, "Y axis value"=0.0, "X axis value"=0.7, "RobotDriveDevRef"=w353) -> ("error out"=w355:errorcluster, "RobotDriveDevRef"=w356:T4)  [unwired: 5 in, 1 out]
            n125 = Subtract(x=w348, y=w347) -> (x-y=w349:dbl)
            "Right Drive Encoder" <- w349
            n126 = Greater?(x=w349, y=198.0) -> (0:w354:bool)
          }
          "Timestamp" <- w341
        }
        frame #7 {
          # "Turns 180"
          n127 = while {
            tunnel: w362 -> [w371]
            tunnel: w361 -> [w370]
            tunnel: [w369] -> w360
            tunnel: [w368] -> w359
            stop <- w363 stop-if-true
            n128 = global read "Robot Global Data.vi" "Real Yaw"() -> (w365:dbl)
            "Real Yaw" <- w365
            n129 = call-poly <vilib>:"WPI_RobotDriveArcadeDrive.vi"("error in (no error)"=w370, "Y axis value"=0.4, "X axis value"=0.0, "RobotDriveDevRef"=w371) -> ("error out"=w368:errorcluster, "RobotDriveDevRef"=w369:T4)  [unwired: 5 in, 1 out]
            n130 = In Range and Coerce(upper limit=170.0, x=w365, lower limit=-170.0) -> (In Range?=w364:bool)  [unwired: 1 out]
            n131 = Not(x=w364) -> (.not. x?=w363:bool)
          }
        }
        frame #8 {
          n132 = call-poly <vilib>:"WPI_RobotDriveArcadeDrive.vi"("error in (no error)"=w374, "Y axis value"=0.0, "X axis value"=0.0, "RobotDriveDevRef"=w375) -> ()  [unwired: 5 in, 3 out]
        }
      }
    }
    frame "top cube-balance" {
      n133 = flat-sequence {
        tunnel: w401 -> [w427]
        tunnel: w402 -> [w426]
        tunnel: w403 -> [w425]
        tunnel: [w427] -> w410
        tunnel: [w426] -> w409
        tunnel: [w425] -> w408
        tunnel: w397 -> [w415]
        tunnel: [w411] -> _
        tunnel: w394 -> [w420]
        tunnel: w396 -> [w417]
        tunnel: w395 -> [w411]
        tunnel: w410 -> [w439]
        tunnel: w409 -> [w437]
        tunnel: w408 -> [w438]
        tunnel: [w431] -> w386
        tunnel: [w430] -> w382
        tunnel: [w429] -> w378
        tunnel: [w478] -> w407
        tunnel: [w477] -> w406
        tunnel: [w472] -> w387
        tunnel: w386 -> [w472]
        tunnel: [w471] -> w383
        tunnel: w382 -> [w471]
        tunnel: [w470] -> w379
        tunnel: w378 -> [w470]
        tunnel: w407 -> [w484]
        tunnel: [w484] -> w405
        tunnel: w406 -> [w483]
        tunnel: [w483] -> w404
        tunnel: [w481] -> w388
        tunnel: w387 -> [w481]
        tunnel: [w480] -> w384
        tunnel: w383 -> [w480]
        tunnel: [w479] -> w380
        tunnel: w379 -> [w479]
        tunnel: w405 -> [w490]
        tunnel: w404 -> [w489]
        tunnel: [w487] -> w389
        tunnel: w388 -> [w487]
        tunnel: [w486] -> w385
        tunnel: w384 -> [w486]
        tunnel: [w485] -> w381
        tunnel: w380 -> [w485]
        tunnel: w389 -> [w499]
        tunnel: w385 -> [w498]
        tunnel: w381 -> [w497]
        tunnel: w400 -> [w531]
        tunnel: w399 -> [w530]
        tunnel: [w532] -> w398
        tunnel: [w531] -> w392
        tunnel: [w530] -> w390
        tunnel: w398 -> [w535]
        tunnel: [w534] -> w393
        tunnel: w392 -> [w534]
        tunnel: [w533] -> w391
        tunnel: w390 -> [w533]
        tunnel: w393 -> [w538]
        tunnel: w391 -> [w537]
        frame #0 {
          n134 = Wait (ms)(milliseconds to wait=u32 30) -> ()  [unwired: 1 out]
          n135 = call <vilib>:"Spark MAX Set Sensor Position.vi"("Sensor Type (Hall Sensor)"=Spark_MAX_Sensor_Type."Hall Sensor", "Position"=0.0, "MotorControlDeviceRef"=w415) -> ("MotorControlDeviceRef"=w414:T5)  [unwired: 7 in, 1 out]
          n136 = call <vilib>:"Spark MAX Set Sensor Position.vi"("Sensor Type (Hall Sensor)"=Spark_MAX_Sensor_Type."Hall Sensor", "Position"=0.0, "MotorControlDeviceRef"=w417) -> ()  [unwired: 7 in, 2 out]
          n137 = call <vilib>:"Spark MAX Get Sensor Position.vi"("MotorControlDevRef in"=w414) -> ()  [unwired: 7 in, 4 out]
          n138 = call <vilib>:"Spark MAX Set Sensor Position.vi"("Sensor Type (Hall Sensor)"=Spark_MAX_Sensor_Type."Hall Sensor", "Position"=0.0, "MotorControlDeviceRef"=w420) -> ()  [unwired: 7 in, 2 out]
          n139 = call <vilib>:"Spark MAX Set Sensor Position.vi"("Sensor Type (Hall Sensor)"=Spark_MAX_Sensor_Type."Hall Sensor", "Position"=0.0, "MotorControlDeviceRef"=w411) -> ()  [unwired: 7 in, 2 out]
        }
        frame #1 {
          n140 = while {
            tunnel: w438 -> [w446]
            tunnel: w437 -> [w445]
            tunnel: w439 -> [w444]
            tunnel: [w441] -> w428
            tunnel: [w443] -> w436
            tunnel: [w442] -> w435
            stop <- w469 stop-if-true
            n141 = global read "Robot Global Data.vi" "Arm Blue"() -> (w449:dbl)
            n142 = global read "Robot Global Data.vi" "Arm Red"() -> (w460:dbl)
            n143 = Subtract(x=145.592, y=w460) -> (x-y=w447:dbl)
            n144 = Subtract(x=67.2, y=w449) -> (x-y=w448:dbl)
            n145 = Multiply(x=w448, y=0.5) -> (x*y=w457:dbl)
            n146 = Multiply(x=w447, y=-0.5) -> (x*y=w456:dbl)
            n147 = In Range and Coerce(upper limit=1.0, x=w448, lower limit=-1.0) -> (In Range?=w468:bool)  [unwired: 1 out]
            n148 = In Range and Coerce(upper limit=1.0, x=w447, lower limit=-1.0) -> (In Range?=w467:bool)  [unwired: 1 out]
            n149 = In Range and Coerce(upper limit=0.2, x=w457, lower limit=-0.2) -> (coerced(x)=w452:dbl)  [unwired: 1 out]
            n150 = In Range and Coerce(upper limit=0.6, x=w456, lower limit=-0.6) -> (coerced(x)=w453:dbl)  [unwired: 1 out]
            n151 = call <vilib>:"WPI_MotorControlSetOutput.vi"("Output"=w452, "MotorControlDevRef"=w445) -> ("MotorControlDevRef"=w441:T5)  [unwired: 7 in, 2 out]
            n152 = call <vilib>:"WPI_MotorControlSetOutput.vi"("Output"=w452, "MotorControlDevRef"=w444) -> ("MotorControlDevRef"=w443:T5)  [unwired: 7 in, 2 out]
            n153 = Wait (ms)(milliseconds to wait=u32 10) -> ()  [unwired: 1 out]
            n154 = call <vilib>:"WPI_MotorControlSetOutput.vi"("Output"=w453, "MotorControlDevRef"=w446) -> ("MotorControlDevRef"=w442:T5)  [unwired: 7 in, 2 out]
            n155 = And(x=w468, y=w467) -> (x .and. y?=w469:bool)
          }
          n156 = call <vilib>:"WPI_MotorControlSetOutput.vi"("Output"=0.0, "MotorControlDevRef"=w435) -> ("MotorControlDevRef"=w431:T5)  [unwired: 7 in, 2 out]
          n157 = call <vilib>:"WPI_MotorControlSetOutput.vi"("Output"=0.0, "MotorControlDevRef"=w428) -> ("MotorControlDevRef"=w430:T5)  [unwired: 7 in, 2 out]
          n158 = call <vilib>:"WPI_MotorControlSetOutput.vi"("Output"=0.0, "MotorControlDevRef"=w436) -> ("MotorControlDevRef"=w429:T5)  [unwired: 7 in, 2 out]
        }
        frame #2 {
          n159 = call <vilib>:"WPI_SolenoidRefNum Registry Get.vi"("refnum name"="Claw") -> ("error out"=w476:errorcluster, "SolenoidDevRef"=w475:T12)  [unwired: 9 in]
          n160 = call-poly <vilib>:"WPI_SolenoidSet.vi"("error in (no error)"=w476, "Value"=WPI_SolenoidValue."On", "SolenoidDevRef"=w475) -> ("error out"=w477:errorcluster, "SolenoidDevRef"=w478:T12)  [unwired: 7 in]
        }
        frame #3 {
          n161 = Wait (ms)(milliseconds to wait=u32 500) -> ()  [unwired: 1 out]
        }
        frame #4 {
          n162 = call-poly <vilib>:"WPI_SolenoidSet.vi"("error in (no error)"=w489, "Value"=WPI_SolenoidValue."Off", "SolenoidDevRef"=w490) -> ()  [unwired: 7 in, 2 out]
        }
        frame #5 {
          # "puts arm in"
          n163 = while {
            tunnel: w499 -> [w506]
            tunnel: w498 -> [w505]
            tunnel: w497 -> [w501]
            tunnel: [w502] -> w496
            tunnel: [w504] -> w495
            tunnel: [w503] -> w494
            stop <- w529 stop-if-true
            n164 = global read "Robot Global Data.vi" "Arm Blue"() -> (w509:dbl)
            n165 = global read "Robot Global Data.vi" "Arm Red"() -> (w520:dbl)
            n166 = Subtract(x=20.0, y=w520) -> (x-y=w507:dbl)
            n167 = Subtract(x=0.0, y=w509) -> (x-y=w508:dbl)
            n168 = Multiply(x=w508, y=0.5) -> (x*y=w517:dbl)
            n169 = Multiply(x=w507, y=-0.5) -> (x*y=w516:dbl)
            n170 = In Range and Coerce(upper limit=1.0, x=w508, lower limit=-1.0) -> (In Range?=w528:bool)  [unwired: 1 out]
            n171 = In Range and Coerce(upper limit=1.0, x=w507, lower limit=-1.0) -> (In Range?=w527:bool)  [unwired: 1 out]
            n172 = In Range and Coerce(upper limit=0.6, x=w517, lower limit=-0.6) -> (coerced(x)=w512:dbl)  [unwired: 1 out]
            n173 = In Range and Coerce(upper limit=0.5, x=w516, lower limit=-0.5) -> (coerced(x)=w513:dbl)  [unwired: 1 out]
            n174 = call <vilib>:"WPI_MotorControlSetOutput.vi"("Output"=w512, "MotorControlDevRef"=w505) -> ("MotorControlDevRef"=w502:T5)  [unwired: 7 in, 2 out]
            n175 = call <vilib>:"WPI_MotorControlSetOutput.vi"("Output"=w512, "MotorControlDevRef"=w501) -> ("MotorControlDevRef"=w504:T5)  [unwired: 7 in, 2 out]
            n176 = call <vilib>:"WPI_MotorControlSetOutput.vi"("Output"=w513, "MotorControlDevRef"=w506) -> ("MotorControlDevRef"=w503:T5)  [unwired: 7 in, 2 out]
            n177 = Wait (ms)(milliseconds to wait=u32 10) -> ()  [unwired: 1 out]
            n178 = And(x=w528, y=w527) -> (x .and. y?=w529:bool)
          }
          n179 = call <vilib>:"WPI_MotorControlSetOutput.vi"("Output"=0.0, "MotorControlDevRef"=w494) -> ()  [unwired: 7 in, 3 out]
          n180 = call <vilib>:"WPI_MotorControlSetOutput.vi"("Output"=0.0, "MotorControlDevRef"=w496) -> ()  [unwired: 7 in, 3 out]
          n181 = call <vilib>:"WPI_MotorControlSetOutput.vi"("Output"=0.0, "MotorControlDevRef"=w495) -> ()  [unwired: 7 in, 3 out]
        }
        frame #6 {
          n182 = Tick Count (ms)() -> (millisecond timer value=w532:u32)
        }
        frame #7 {
          n183 = call "Balance.vi"("Start Time"=w535, "Boolean"=TRUE) -> ()  [unwired: 10 in]
        }
        frame #8 {
          n184 = call-poly <vilib>:"WPI_RobotDriveArcadeDrive.vi"("error in (no error)"=w537, "Y axis value"=0.0, "X axis value"=0.0, "RobotDriveDevRef"=w538) -> ()  [unwired: 5 in, 3 out]
        }
      }
    }
    frame "top cube" {
      n185 = flat-sequence {
        tunnel: w564 -> [w585]
        tunnel: w565 -> [w584]
        tunnel: w566 -> [w583]
        tunnel: [w585] -> w559
        tunnel: [w573] -> w554
        tunnel: [w584] -> w553
        tunnel: [w583] -> w552
        tunnel: w551 -> [w570]
        tunnel: w550 -> [w580]
        tunnel: w549 -> [w577]
        tunnel: w548 -> [w574]
        tunnel: [w572] -> w543
        tunnel: w559 -> [w596]
        tunnel: [w595] -> w555
        tunnel: w554 -> [w595]
        tunnel: w553 -> [w593]
        tunnel: w552 -> [w594]
        tunnel: [w592] -> w544
        tunnel: w543 -> [w592]
        tunnel: [w627] -> w556
        tunnel: w555 -> [w627]
        tunnel: [w626] -> w545
        tunnel: w544 -> [w626]
        tunnel: [w635] -> w563
        tunnel: [w634] -> w561
        tunnel: [w633] -> w557
        tunnel: w556 -> [w633]
        tunnel: [w632] -> w546
        tunnel: w545 -> [w632]
        tunnel: w563 -> [w640]
        tunnel: [w640] -> w562
        tunnel: w561 -> [w639]
        tunnel: [w639] -> w560
        tunnel: [w638] -> w558
        tunnel: w557 -> [w638]
        tunnel: [w637] -> w547
        tunnel: w546 -> [w637]
        tunnel: w562 -> [w644]
        tunnel: w560 -> [w643]
        tunnel: w558 -> [_]
        tunnel: w547 -> [_]
        tunnel: [w642] -> w542
        tunnel: w541 -> [w642]
        tunnel: w542 -> [w645]
        frame #0 {
          n186 = Wait (ms)(milliseconds to wait=u32 30) -> ()  [unwired: 1 out]
          n187 = call <vilib>:"Spark MAX Set Sensor Position.vi"("Sensor Type (Hall Sensor)"=Spark_MAX_Sensor_Type."Hall Sensor", "Position"=0.0, "MotorControlDeviceRef"=w570) -> ("MotorControlDeviceRef"=w569:T5)  [unwired: 7 in, 1 out]
          n188 = call <vilib>:"Spark MAX Set Sensor Position.vi"("Sensor Type (Hall Sensor)"=Spark_MAX_Sensor_Type."Hall Sensor", "Position"=0.0, "MotorControlDeviceRef"=w574) -> ()  [unwired: 7 in, 2 out]
          n189 = call <vilib>:"Spark MAX Get Sensor Position.vi"("MotorControlDevRef in"=w569) -> ("Sensor Position"=w572:dbl, "MotorControlDevRef out"=w573:T5)  [unwired: 7 in, 2 out]
          n190 = call <vilib>:"Spark MAX Set Sensor Position.vi"("Sensor Type (Hall Sensor)"=Spark_MAX_Sensor_Type."Hall Sensor", "Position"=0.0, "MotorControlDeviceRef"=w577) -> ()  [unwired: 7 in, 2 out]
          n191 = call <vilib>:"Spark MAX Set Sensor Position.vi"("Sensor Type (Hall Sensor)"=Spark_MAX_Sensor_Type."Hall Sensor", "Position"=0.0, "MotorControlDeviceRef"=w580) -> ()  [unwired: 7 in, 2 out]
        }
        frame #1 {
          n192 = while {
            tunnel: w594 -> [w602]
            tunnel: w593 -> [w601]
            tunnel: w596 -> [w600]
            tunnel: [w597] -> w591
            tunnel: [w599] -> w590
            tunnel: [w598] -> w589
            stop <- w625 stop-if-true
            n193 = global read "Robot Global Data.vi" "Arm Blue"() -> (w605:dbl)
            n194 = global read "Robot Global Data.vi" "Arm Red"() -> (w616:dbl)
            n195 = Subtract(x=145.592, y=w616) -> (x-y=w603:dbl)
            n196 = Subtract(x=67.2, y=w605) -> (x-y=w604:dbl)
            n197 = Multiply(x=w604, y=0.5) -> (x*y=w613:dbl)
            n198 = Multiply(x=w603, y=-0.5) -> (x*y=w612:dbl)
            n199 = In Range and Coerce(upper limit=1.0, x=w604, lower limit=-1.0) -> (In Range?=w624:bool)  [unwired: 1 out]
            n200 = In Range and Coerce(upper limit=1.0, x=w603, lower limit=-1.0) -> (In Range?=w623:bool)  [unwired: 1 out]
            n201 = In Range and Coerce(upper limit=0.2, x=w613, lower limit=-0.2) -> (coerced(x)=w608:dbl)  [unwired: 1 out]
            n202 = In Range and Coerce(upper limit=0.6, x=w612, lower limit=-0.6) -> (coerced(x)=w609:dbl)  [unwired: 1 out]
            n203 = call <vilib>:"WPI_MotorControlSetOutput.vi"("Output"=w608, "MotorControlDevRef"=w601) -> ("MotorControlDevRef"=w597:T5)  [unwired: 7 in, 2 out]
            n204 = call <vilib>:"WPI_MotorControlSetOutput.vi"("Output"=w608, "MotorControlDevRef"=w600) -> ("MotorControlDevRef"=w599:T5)  [unwired: 7 in, 2 out]
            n205 = call <vilib>:"WPI_MotorControlSetOutput.vi"("Output"=w609, "MotorControlDevRef"=w602) -> ("MotorControlDevRef"=w598:T5)  [unwired: 7 in, 2 out]
            n206 = And(x=w624, y=w623) -> (x .and. y?=w625:bool)
          }
          n207 = call <vilib>:"WPI_MotorControlSetOutput.vi"("Output"=0.0, "MotorControlDevRef"=w589) -> ()  [unwired: 7 in, 3 out]
          n208 = call <vilib>:"WPI_MotorControlSetOutput.vi"("Output"=0.0, "MotorControlDevRef"=w591) -> ()  [unwired: 7 in, 3 out]
          n209 = call <vilib>:"WPI_MotorControlSetOutput.vi"("Output"=0.0, "MotorControlDevRef"=w590) -> ()  [unwired: 7 in, 3 out]
        }
        frame #2 {
        }
        frame #3 {
          n210 = call <vilib>:"WPI_SolenoidRefNum Registry Get.vi"("refnum name"="Claw") -> ("error out"=w631:errorcluster, "SolenoidDevRef"=w630:T12)  [unwired: 9 in]
          n211 = call-poly <vilib>:"WPI_SolenoidSet.vi"("error in (no error)"=w631, "Value"=WPI_SolenoidValue."On", "SolenoidDevRef"=w630) -> ("error out"=w634:errorcluster, "SolenoidDevRef"=w635:T12)  [unwired: 7 in]
        }
        frame #4 {
          n212 = Wait (ms)(milliseconds to wait=u32 500) -> ()  [unwired: 1 out]
        }
        frame #5 {
          n213 = call-poly <vilib>:"WPI_SolenoidSet.vi"("error in (no error)"=w643, "Value"=WPI_SolenoidValue."Off", "SolenoidDevRef"=w644) -> ()  [unwired: 7 in, 2 out]
        }
        frame #6 {
          n214 = call-poly <vilib>:"WPI_RobotDriveArcadeDrive.vi"("Y axis value"=0.0, "X axis value"=0.0, "RobotDriveDevRef"=w645) -> ()  [unwired: 6 in, 3 out]
        }
      }
    }
    frame "Balance" {
      # "You can put your main auto here, or you can right-click on the case and make any\nother frame be the default case."
      # "This is the frame that will execute if no selection is made, or if it is not recognized"
      n215 = flat-sequence {
        tunnel: [w649] -> w648
        tunnel: w648 -> [w651]
        frame #0 {
          n216 = Tick Count (ms)() -> (millisecond timer value=w649:u32)
        }
        frame #1 {
          n217 = call "Balance.vi"("Start Time"=w651, "Boolean"=TRUE) -> ()  [unwired: 10 in]
        }
      }
    }
    frame "Drive Straight" {
      n218 = flat-sequence {
        tunnel: [w657] -> w654
        tunnel: w653 -> [w657]
        tunnel: [w663] -> w656
        tunnel: [w662] -> w655
        tunnel: w654 -> [w660]
        tunnel: w652 -> [w659]
        tunnel: w656 -> [w676]
        tunnel: w655 -> [w675]
        frame #0 {
          # "Creates the starting angle"
          n219 = global read "Robot Global Data.vi" "yaw"() -> (w658:dbl)
          n220 = global write "Robot Global Data.vi" "Gyro Starting Value in our match"(w658) -> ()
        }
        frame #1 {
          n221 = Tick Count (ms)() -> (millisecond timer value=w661:u32)
          n222 = while {
            tunnel: [w673] -> w663
            tunnel: [w672] -> w662
            tunnel: w661 -> [w670]
            tunnel: w660 -> [w665]
            tunnel: w659 -> [w664]
            stop <- w666 stop-if-true
            n223 = call "Drive straight.vi"("Start Time"=w670, "Length(seconds)"=6.0, "Desired angle"=0.0) -> ("Complete or not"=w666:bool, "X Power"=w667:dbl)  [unwired: 7 in]
            n224 = Wait (ms)(milliseconds to wait=u32 10) -> ()  [unwired: 1 out]
            n225 = call-poly <vilib>:"WPI_RobotDriveArcadeDrive.vi"("error in (no error)"=w664, "Y axis value"=-0.55, "X axis value"=w667, "RobotDriveDevRef"=w665) -> ("error out"=w672:errorcluster, "RobotDriveDevRef"=w673:T4)  [unwired: 5 in, 1 out]
          }
        }
        frame #2 {
          n226 = call-poly <vilib>:"WPI_RobotDriveArcadeDrive.vi"("error in (no error)"=w675, "Y axis value"=0.0, "X axis value"=0.0, "RobotDriveDevRef"=w676) -> ()  [unwired: 5 in, 3 out]
        }
      }
    }
    frame "Test Balance" {
      n227 = flat-sequence {
        tunnel: w683 -> [w725]
        tunnel: w684 -> [w724]
        tunnel: w685 -> [w723]
        tunnel: [w725] -> w706
        tunnel: [w715] -> w705
        tunnel: [w724] -> w704
        tunnel: [w723] -> w703
        tunnel: [w709] -> _
        tunnel: [w708] -> _
        tunnel: w688 -> [w716]
        tunnel: [w714] -> w702
        tunnel: w689 -> [w709]
        tunnel: w687 -> [w708]
        tunnel: w686 -> [w707]
        tunnel: w706 -> [w736]
        tunnel: [w735] -> w701
        tunnel: w705 -> [w735]
        tunnel: w704 -> [w733]
        tunnel: w703 -> [w734]
        tunnel: [w732] -> w700
        tunnel: w702 -> [w732]
        tunnel: [w767] -> w699
        tunnel: w701 -> [w767]
        tunnel: [w766] -> w698
        tunnel: w700 -> [w766]
        tunnel: [w775] -> w697
        tunnel: [w774] -> w696
        tunnel: [w773] -> w695
        tunnel: w699 -> [w773]
        tunnel: [w772] -> w694
        tunnel: w698 -> [w772]
        tunnel: w697 -> [w780]
        tunnel: [w780] -> w693
        tunnel: w696 -> [w779]
        tunnel: [w779] -> w692
        tunnel: [w778] -> w691
        tunnel: w695 -> [w778]
        tunnel: [w777] -> w690
        tunnel: w694 -> [w777]
        tunnel: w693 -> [w783]
        tunnel: w692 -> [w782]
        tunnel: w691 -> [_]
        tunnel: w690 -> [_]
        tunnel: w682 -> [w787]
        tunnel: w681 -> [w786]
        tunnel: [w785] -> w680
        tunnel: [w784] -> w679
        tunnel: w680 -> [w800]
        tunnel: w679 -> [w799]
        frame #0 {
          n228 = Wait (ms)(milliseconds to wait=u32 30) -> ()  [unwired: 1 out]
          n229 = call <vilib>:"Spark MAX Set Sensor Position.vi"("Sensor Type (Hall Sensor)"=Spark_MAX_Sensor_Type."Hall Sensor", "Position"=0.0, "MotorControlDeviceRef"=w709) -> ("MotorControlDeviceRef"=w712:T5)  [unwired: 7 in, 1 out]
          n230 = call <vilib>:"Spark MAX Set Sensor Position.vi"("Sensor Type (Hall Sensor)"=Spark_MAX_Sensor_Type."Hall Sensor", "Position"=0.0, "MotorControlDeviceRef"=w716) -> ()  [unwired: 7 in, 2 out]
          n231 = call <vilib>:"Spark MAX Get Sensor Position.vi"("MotorControlDevRef in"=w712) -> ("Sensor Position"=w714:dbl, "MotorControlDevRef out"=w715:T5)  [unwired: 7 in, 2 out]
          n232 = call <vilib>:"Spark MAX Set Sensor Position.vi"("Sensor Type (Hall Sensor)"=Spark_MAX_Sensor_Type."Hall Sensor", "Position"=0.0, "MotorControlDeviceRef"=w707) -> ()  [unwired: 7 in, 2 out]
          n233 = call <vilib>:"Spark MAX Set Sensor Position.vi"("Sensor Type (Hall Sensor)"=Spark_MAX_Sensor_Type."Hall Sensor", "Position"=0.0, "MotorControlDeviceRef"=w708) -> ()  [unwired: 7 in, 2 out]
        }
        frame #1 {
          n234 = while {
            tunnel: w734 -> [w742]
            tunnel: w733 -> [w741]
            tunnel: w736 -> [w740]
            tunnel: [w737] -> w731
            tunnel: [w739] -> w730
            tunnel: [w738] -> w729
            stop <- w765 stop-if-true
            n235 = global read "Robot Global Data.vi" "Arm Blue"() -> (w745:dbl)
            n236 = global read "Robot Global Data.vi" "Arm Red"() -> (w756:dbl)
            n237 = Subtract(x=145.592, y=w756) -> (x-y=w743:dbl)
            n238 = Subtract(x=67.2, y=w745) -> (x-y=w744:dbl)
            n239 = Multiply(x=w744, y=0.5) -> (x*y=w753:dbl)
            n240 = Multiply(x=w743, y=-0.5) -> (x*y=w752:dbl)
            n241 = In Range and Coerce(upper limit=1.0, x=w744, lower limit=-1.0) -> (In Range?=w764:bool)  [unwired: 1 out]
            n242 = In Range and Coerce(upper limit=1.0, x=w743, lower limit=-1.0) -> (In Range?=w763:bool)  [unwired: 1 out]
            n243 = In Range and Coerce(upper limit=0.2, x=w753, lower limit=-0.2) -> (coerced(x)=w748:dbl)  [unwired: 1 out]
            n244 = In Range and Coerce(upper limit=0.6, x=w752, lower limit=-0.6) -> (coerced(x)=w749:dbl)  [unwired: 1 out]
            n245 = call <vilib>:"WPI_MotorControlSetOutput.vi"("Output"=w748, "MotorControlDevRef"=w741) -> ("MotorControlDevRef"=w737:T5)  [unwired: 7 in, 2 out]
            n246 = call <vilib>:"WPI_MotorControlSetOutput.vi"("Output"=w748, "MotorControlDevRef"=w740) -> ("MotorControlDevRef"=w739:T5)  [unwired: 7 in, 2 out]
            n247 = call <vilib>:"WPI_MotorControlSetOutput.vi"("Output"=w749, "MotorControlDevRef"=w742) -> ("MotorControlDevRef"=w738:T5)  [unwired: 7 in, 2 out]
            n248 = And(x=w764, y=w763) -> (x .and. y?=w765:bool)
          }
          n249 = call <vilib>:"WPI_MotorControlSetOutput.vi"("Output"=0.0, "MotorControlDevRef"=w729) -> ()  [unwired: 7 in, 3 out]
          n250 = call <vilib>:"WPI_MotorControlSetOutput.vi"("Output"=0.0, "MotorControlDevRef"=w731) -> ()  [unwired: 7 in, 3 out]
          n251 = call <vilib>:"WPI_MotorControlSetOutput.vi"("Output"=0.0, "MotorControlDevRef"=w730) -> ()  [unwired: 7 in, 3 out]
        }
        frame #2 {
        }
        frame #3 {
          n252 = call <vilib>:"WPI_SolenoidRefNum Registry Get.vi"("refnum name"="Claw") -> ("error out"=w771:errorcluster, "SolenoidDevRef"=w770:T12)  [unwired: 9 in]
          n253 = call-poly <vilib>:"WPI_SolenoidSet.vi"("error in (no error)"=w771, "Value"=WPI_SolenoidValue."On", "SolenoidDevRef"=w770) -> ("error out"=w774:errorcluster, "SolenoidDevRef"=w775:T12)  [unwired: 7 in]
        }
        frame #4 {
          n254 = Wait (ms)(milliseconds to wait=u32 500) -> ()  [unwired: 1 out]
        }
        frame #5 {
          n255 = call "arm back.vi"() -> ()  [unwired: 12 in]
          n256 = call-poly <vilib>:"WPI_SolenoidSet.vi"("error in (no error)"=w782, "Value"=WPI_SolenoidValue."Off", "SolenoidDevRef"=w783) -> ()  [unwired: 7 in, 2 out]
        }
        frame #6 {
          n257 = while {
            shift-right: [w795] -> w785
            shift-left: w787 -> [w798]
            shift-right: [w796] -> w784
            shift-left: w786 -> [w797]
            stop <- w790 stop-if-true
            n258 = global read "Robot Global Data.vi" "Pitch"() -> (w792:dbl)
            n259 = call-poly <vilib>:"WPI_RobotDriveArcadeDrive.vi"("error in (no error)"=w797, "Y axis value"=0.0 ("X axis value"), "X axis value"=0.55 ("Y axis value"), "RobotDriveDevRef"=w798) -> ("error out"=w796:errorcluster, "RobotDriveDevRef"=w795:T4)  [unwired: 5 in, 1 out]
            n260 = In Range and Coerce(upper limit=10.0, x=w792, lower limit=-10.0 ("y")) -> (In Range?=w793:bool)  [unwired: 1 out]
            n261 = Not(x=w793) -> (.not. x?=w790:bool)
          }
        }
        frame #7 {
          n262 = while {
            tunnel: w799 -> [w805]
            tunnel: w800 -> [w804]
            stop <- FALSE stop-if-true
            n263 = call "Derivative balance.vi"() -> ("Motor Power"=w802:dbl)  [unwired: 11 in]
            n264 = Negate(x=w802) -> (-x=w801:dbl)
            n265 = call-poly <vilib>:"WPI_RobotDriveArcadeDrive.vi"("error in (no error)"=w805, "Y axis value"=0.0 ("X axis value"), "X axis value"=w801, "RobotDriveDevRef"=w804) -> ()  [unwired: 5 in, 3 out]
          }
        }
      }
    }
    frame Default {
    }
  }
